vi "Read data.vi"(8 "error in (no error)":errorcluster, 11 "ZM-PC-EP-error_package in":refnum<class "ZM-PC-EP-error_package.lvclass">) -> (0 "error out":errorcluster, 2 "ZM-PC-EP-DATA":T1, 3 "ZM-PC-EP-error_package out":refnum<class "ZM-PC-EP-error_package.lvclass">)   [LabVIEW 2020, in "ZM-PC-packages.lvlib" / "ZM-PC-EP-error_package.lvclass"]
doc: "Reads one field of this class's private data. Generated by lvai_create_accessors from the class private data control."
uses:
  ZM-PC-EP-error_package.lvclass
  ZM-PC-EP-error_package.lvclass/ZM-PC-EP-error_package.ctl
  ZM-PC-EP-DATA.ctl
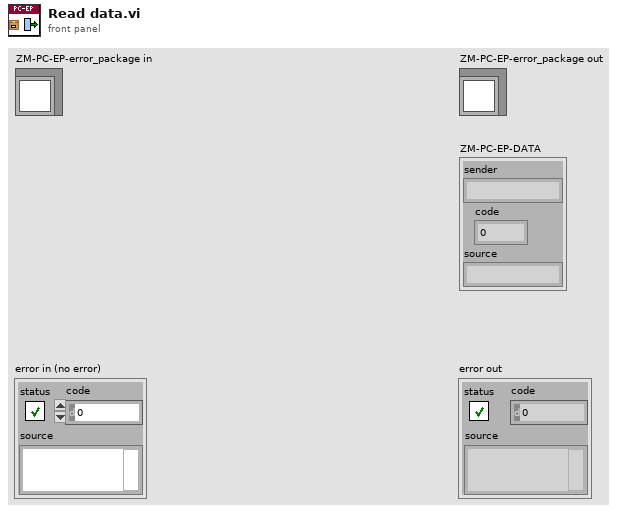
[diagram p1: front panel]
types:
  T1 = typedef "ZM-PC-packages.lvlib/ZM-PC-EP-error_package.lvclass/ZM-PC-EP-DATA.ctl" = cluster{"sender":string, "code":i32, "source":string}
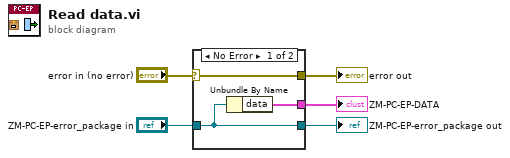
[diagram p0: block diagram]
diagram:
  n1 = case shown="No Error" "error in (no error)" {
    selector: "error in (no error)" -> [w8 w9]
    tunnel: [w8 w9] -> w4
    tunnel: [w7 w10] -> w2
    tunnel: "ZM-PC-EP-error_package in" -> [w7 w10]
    tunnel: [w6 _] -> w1
    frame No Error {
      n2 = Unbundle By Name(w7) -> ("data"=w6:T1)
    }
    frame Error {
    }
  }
  "error out" <- w4
  "ZM-PC-EP-error_package out" <- w2
  "ZM-PC-EP-DATA" <- w1
